vi "work1_GetOrder and Cook.vi"() -> ()   [LabVIEW 2026]
panel:
  out "Client Counter":i32
  in  "stop":bool
  out "Order ID":i32
  in  "ID":i32
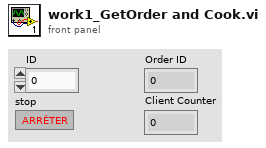
[diagram p1: front panel]
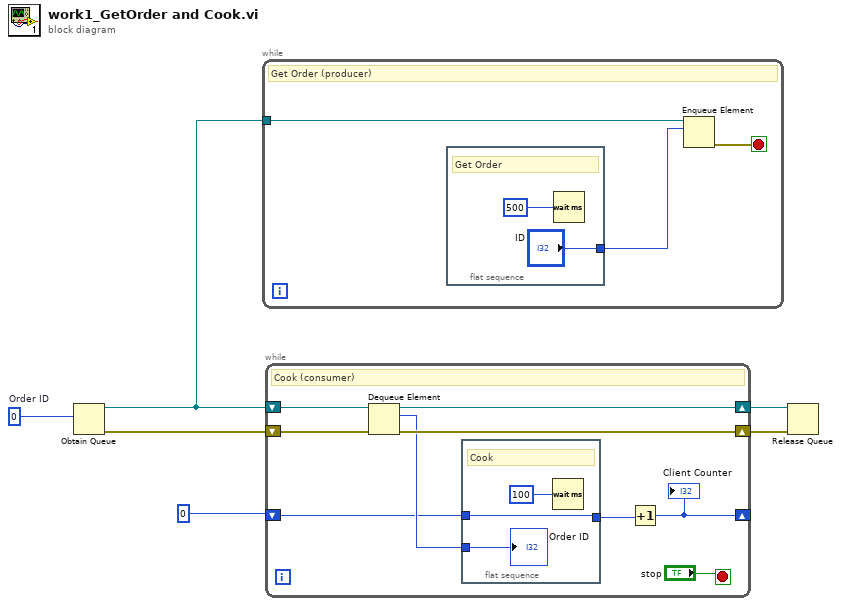
[diagram p0: block diagram]
diagram:
  w2 = 0  # Order ID
  n1 = Obtain Queue(element data type=w2) -> (queue out=w3:refnum<queue>, error out=w6:errorcluster)  [unwired: 4 in, 1 out]
  n2 = while {
    tunnel: w3 -> [w9]
    stop <- w8 stop-if-true
    # "Get Order (producer)"
    n3 = flat-sequence {
      tunnel: ["ID"] -> w7
      frame #0 {
        # "Get Order"
        n4 = Wait (ms)(milliseconds to wait=500) -> ()  [unwired: 1 out]
      }
    }
    n5 = Enqueue Element(queue=w9, element=w7) -> (error out=w8:errorcluster)  [unwired: 2 in, 2 out]
  }
  n6 = while {
    shift-right: [w18] -> w4
    shift-left: w6 -> [w20]
    shift-right: [w19] -> w5
    shift-left: w3 -> [w17]
    shift-right: [w12] -> _
    shift-left: 0 -> [w14]
    stop <- "stop" stop-if-true
    # "Cook (consumer)"
    n7 = Dequeue Element(queue=w17, error in (no error)=w20) -> (queue out=w19:refnum<queue>, element=w16:i32, error out=w18:errorcluster)  [unwired: 1 in, 1 out]
    n8 = flat-sequence {
      tunnel: w16 -> [w22]
      tunnel: w14 -> [w21]
      tunnel: [w21] -> w13
      frame #0 {
        # "Cook"
        n9 = Wait (ms)(milliseconds to wait=100) -> ()  [unwired: 1 out]
        "Order ID" <- w22
      }
    }
    n10 = Increment(x=w13) -> (x+1=w12:i32)
    "Client Counter" <- w12
  }
  n11 = Release Queue(queue=w5, error in (no error)=w4) -> ()  [unwired: 1 in, 3 out]
